vi "RemoteVI Close Clients.vi"(0 "clients":T2(array[cluster]), 5 "pending":T1(array[cluster])) -> ()   [LabVIEW 2020, in "RemoteVI.lvlib"]
doc: "Ends every connection when the server stops: each client gets a WebSocket close frame 1001 (going away, 500 ms write timeout) and is closed; each pending connection (not answered yet) is closed. Connections are TCP refnums type-cast to U32."
uses:
  RemoteVI.lvlib
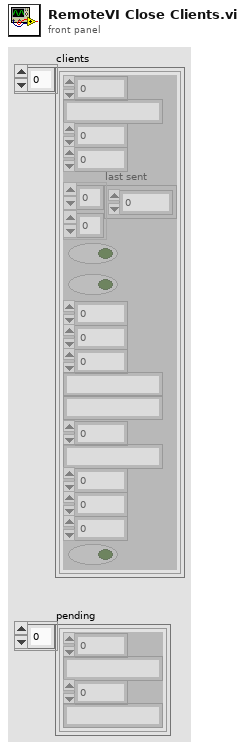
[diagram p1: front panel]
types:
  T1 = cluster{"connection":u32, "head":string, "accepted":u32, "address":string}[]
  T2 = cluster{"connection":u32, "rx buffer":string, "seq":u32, "acked":u32, "last sent":u32[][], "tracking":bool, "closed":bool, "mods":u8, "mods set":u8, "popup since":u32, "windows sent":string, "window frames":cluster{"id":u64, "pixels":u32[][]}[], "key window":u64, "address":string, "since":dbl, "last input":dbl, "bytes":dbl, "view only":bool}[]
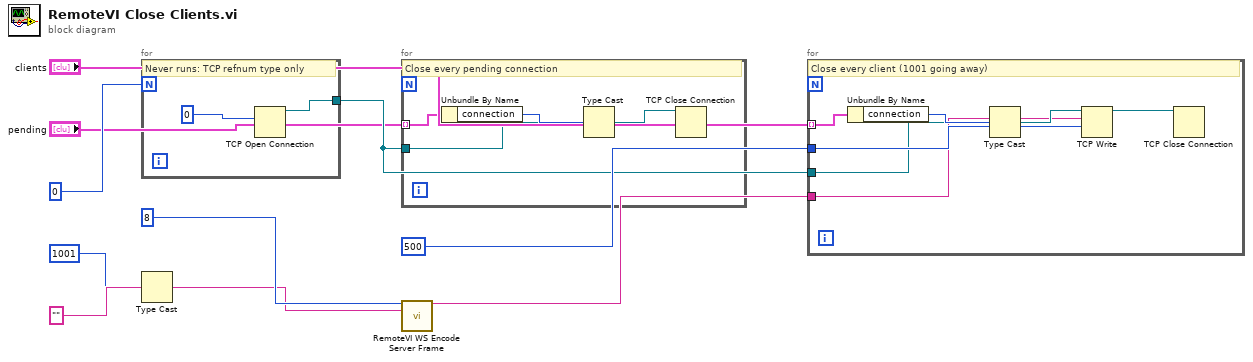
[diagram p0: block diagram]
diagram:
  n1 = for {
    N: 0 -> [_]
    tunnel: [w12] -> w4
    # "Never runs: TCP refnum type only"
    n2 = TCP Open Connection(remote port or service name=u16 0) -> (connection ID=w12:refnum<k5>)  [unwired: 4 in, 1 out]
  }
  n3 = Type Cast(type="", x=u16 1001) -> (*(type *) &x=w7:string)
  n4 = for {
    tunnel: "pending" -> [w13] mode=indexing
    tunnel: w4 -> [w14]
    # "Close every pending connection"
    n5 = Unbundle By Name(w13) -> ("connection"=w15:u32)
    n6 = Type Cast(type=w14, x=w15) -> (*(type *) &x=w16:refnum<k5>)
    n7 = TCP Close Connection(connection ID=w16) -> ()  [unwired: 2 in, 2 out]
  }
  n8 = call "RemoteVI WS Encode Server Frame.vi"("opcode"=u8 8, "payload"=w7) -> ("frame"=w9:string)  [unwired: 13 in]
  n9 = for {
    tunnel: "clients" -> [w17] mode=indexing
    tunnel: 500 -> [w20]
    tunnel: w4 -> [w18]
    tunnel: w9 -> [w19]
    # "Close every client (1001 going away)"
    n10 = Unbundle By Name(w17) -> ("connection"=w21:u32)
    n11 = Type Cast(type=w18, x=w21) -> (*(type *) &x=w22:refnum<k5>)
    n12 = TCP Write(connection ID=w22, data in=w19, 9:w20) -> (connection ID out=w23:refnum<k5>)  [unwired: 1 in, 2 out]
    n13 = TCP Close Connection(connection ID=w23) -> ()  [unwired: 2 in, 2 out]
  }
